vi "Core Read U8 External FIFO.vi"(8 "error in (no error)":errorcluster, 9 "Timeout (ms)":i32, 11 "CIFFIFO in":refnum<class "CIF_Iceoryx_PCAP_Universal.lvclass">) -> (0 "error out":errorcluster, 1 "timed out?":bool, 3 "CIFFIFO out":refnum<class "CIF_Iceoryx_PCAP_Universal.lvclass">)   [LabVIEW 2021, in "CIF_Iceoryx_PCAP_Universal.lvclass"]
uses:
  CIF_Iceoryx_PCAP_Universal.lvclass
  CIF_Iceoryx_PCAP_Universal.lvclass/CIF_Iceoryx_PCAP_Universal.ctl
  ChannelCommon/typedef/Direction.ctl
  ChannelCommon/ChannelCommon.lvlib
  ChannelCommon/typedef/Channel State.ctl
  CIFChannels/CIFChannels.lvclass
  e703c505-0034-46a9-8989-21c0de27793f.vi
  768488f4-e6df-4560-a449-a64b33b49031.vi
  <vilib>/CIF Foundation/CIF Iceoryx/Iceoryx.lvlib
  D:/dev/Packages/CIF_Channels_Core/src/Iceorxy_Channels/CIF_Iceoryx_Chan/CIF_Iceoryx_Chn.lvclass
  D:/dev/Packages/CIF_Channels_Core/src/CIFChannels/CIFChannels.lvclass
  D:/dev/Packages/CIF_Channels_Core/src/Iceorxy_Channels/PCAP_Universal/CIF_Iceoryx_PCAP_Universal.lvclass
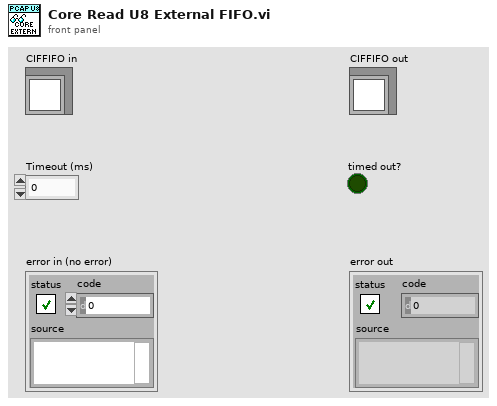
[diagram p1: front panel]
types:
  T1 = typedef "ChannelCommon.lvlib/Channel State.ctl" = enum8{"Creating", "Disconnected", "Connecting", "Connected", "Destroyed"}
  T2 = typedef "ChannelCommon.lvlib/Direction.ctl" = enum8{"Publisher", "Subscriber"}
  T3 = typedef "Iceoryx.lvlib/CIF Subscriber Refnum.ctl" = cluster{"refnum":u64, "CIF Sub":enum8{"cifsub"}}
  T4 = typedef "ChannelCommon.lvlib/FIFO Header.ctl" = cluster{"Length":u64, "T0":i64, "T_Out":i64, "T_Tx":i64, "Ctr":u64, "ClockID":u8}
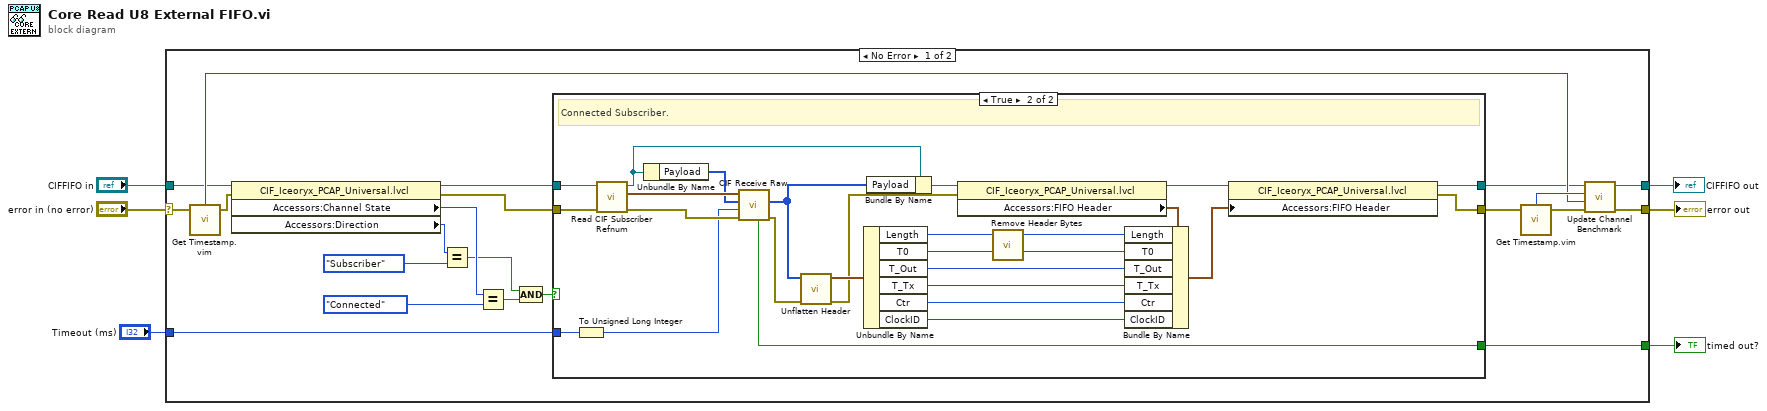
[diagram p0: block diagram]
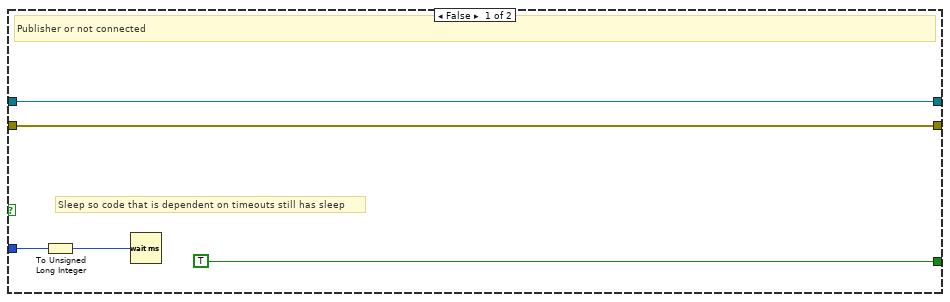
[diagram p2: hidden frame]
diagram:
  n1 = case shown="No Error" "error in (no error)" {
    selector: "error in (no error)" -> [w9 w60]
    tunnel: [w15 w60] -> w1
    tunnel: [w16 w59] -> w2
    tunnel: "CIFFIFO in" -> [w8 w59]
    tunnel: [w27 _] -> w3
    tunnel: "Timeout (ms)" -> [w17 _]
    frame No Error {
      n2 = call "Get Timestamp.vim"("Anything in"=w9) -> ("Time (ns)"=w13:i64, "Anything out"=w7:errorcluster)  [unwired: 2 in]
      n3 = property class="CIF_Iceoryx_PCAP_Universal.lvcl"(reference=w8, error in=w7) -> (reference out=w26:refnum<class "CIF_Iceoryx_PCAP_Universal.lvclass">, error out=w25:errorcluster, "Accessors:Channel State"=w22:T1, "Accessors:Direction"=w24:T2)
      n4 = Equal?(x=w24, y=Direction."Subscriber") -> (x = y?=w18:bool)
      n5 = Equal?(x=w22, y=Channel_State."Connected") -> (x = y?=w20:bool)
      n6 = Compound Arithmetic op=AND(w18, w20) -> (w19:bool)
      n7 = case shown="True" w19 {
        tunnel: [TRUE ("timeout out") w51] -> w27
        tunnel: w25 -> [w31 w58]
        tunnel: w26 -> [w32 w55]
        tunnel: [w32 w40] -> w11
        tunnel: [w31 w39] -> w10
        tunnel: w17 -> [w29 w53]
        frame False {
          # "Sleep so code that is dependent on timeouts still has sleep"
          # "Publisher or not connected"
          n8 = To Unsigned Long Integer(number=w29) -> (unsigned 32bit integer=w28:u32)
          n9 = Wait (ms)(milliseconds to wait=w28) -> ()  [unwired: 1 out]
        }
        frame True {
          # "Connected Subscriber."
          n10 = To Unsigned Long Integer(number=w53) -> (unsigned 32bit integer=w52:u32)
          n11 = call "Read CIF Subscriber Refnum.vi"("error in (no error)"=w58, "CIF_Iceoryx_PCAP_Universal in"=w55) -> ("error out"=w56:errorcluster, "CIF Subscriber Refnum"=w57:T3, "CIF_Iceoryx_PCAP_Universal out"=w50:refnum<class "CIF_Iceoryx_PCAP_Universal.lvclass">)  [unwired: 7 in]
          n12 = Unbundle By Name(w50) -> ("Payload"=w54:u8[])
          n13 = call <vilib>:"CIF Receive Raw.vi"("error in (no error)"=w56, "Timoeut ms"=w52, "Data In"=w54, "Subscriber Reference"=w57) -> ("error out"=w34:errorcluster, "Data Out"=w36:u8[], "Timeout"=w51:bool)  [unwired: 3 in, 2 out]
          n14 = call "Unflatten Header.vi"("error in (no error)"=w34, "Flattened Data in"=w36) -> ("error out"=w33:errorcluster, "Header out"=w35:T4)  [unwired: 7 in, 1 out]
          n15 = Unbundle By Name(w35) -> ("Length"=w38:u64, "T0"=w47:i64, "T_Out"=w46:i64, "T_Tx"=w45:i64, "Ctr"=w44:u64, "ClockID"=w43:u8)
          n16 = Bundle By Name(cluster=w50, "Payload"=w36) -> (w49:refnum<class "CIF_Iceoryx_PCAP_Universal.lvclass">)
          n17 = property class="CIF_Iceoryx_PCAP_Universal.lvcl"(reference=w49, error in=w33) -> (reference out=w41:refnum<class "CIF_Iceoryx_PCAP_Universal.lvclass">, "Accessors:FIFO Header"=w48:T4)  [unwired: 1 out]
          n18 = call "Remove Header Bytes.vi"("Bytes/Msg with header"=w38) -> ("Bytes/Msg without header"=w37:u64)  [unwired: 3 in]
          n19 = Bundle By Name(cluster=w48, "Length"=w37, "T0"=w47, "T_Out"=w46, "T_Tx"=w45, "Ctr"=w44, "ClockID"=w43) -> (w42:T4)
          n20 = property class="CIF_Iceoryx_PCAP_Universal.lvcl"(reference=w41, "Accessors:FIFO Header"=w42) -> (reference out=w40:refnum<class "CIF_Iceoryx_PCAP_Universal.lvclass">, error out=w39:errorcluster)  [unwired: 1 in]
        }
      }
      n21 = call "Get Timestamp.vim"("Anything in"=w10) -> ("Time (ns)"=w14:i64, "Anything out"=w12:errorcluster)  [unwired: 2 in]
      n22 = call "Update Channel Benchmark.vi"("error in (no error)"=w12, "X0"=w13, "X1"=w14, "CIFChannels in"=w11) -> ("error out"=w15:errorcluster, "CIFChannels out"=w16:refnum<class "CIF_Iceoryx_PCAP_Universal.lvclass">)  [unwired: 6 in]
    }
    frame Error {
    }
  }
  "error out" <- w1
  "timed out?" <- w3
  "CIFFIFO out" <- w2
